vi "Read Index.vi"(8 "error in (no error)":errorcluster, 11 "NT Enum in":refnum<class "NT Enum.lvclass">) -> (0 "error out":errorcluster, 2 "index":i32, 3 "NT Enum out":refnum<class "NT Enum.lvclass">)   [LabVIEW 2020, in "PV Access.lvlib" / "PV Data.lvlib" / "NT Enum.lvclass"]
uses:
  NT Enum.lvclass
  NT Enum.lvclass/NT Enum.ctl
  9e0b9964-89ef-45f4-810c-f4d4147585a8.vi
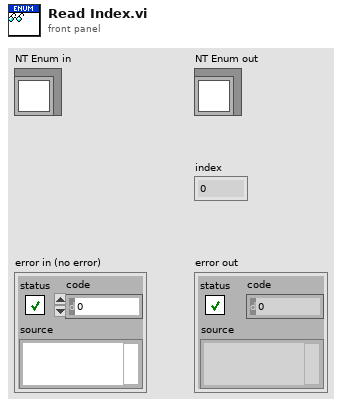
[diagram p1: front panel]
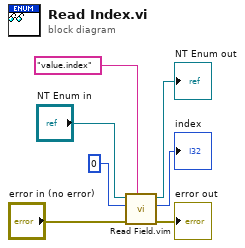
[diagram p0: block diagram]
diagram:
  n1 = call "Read Field.vim"("field"="value.index", "error in"="error in (no error)", "default value"=0, "Base Interface in"="NT Enum in") -> ("error out"=→"error out":errorcluster, "value"=→"index":i32, "Base Interface out"=→"NT Enum out":refnum<class "NT Enum.lvclass">)  [unwired: 5 in]
